vi "VIH UI - Append Control Rules.vi"(9 "Position Index (-1)":i32=-1, 10 "Ctrl Rules (new)":T1[](array[typedef]), 11 "Ctrl Rules (existing)":T1[](array[typedef])) -> (1 "Indices":i32[](array[numeric]), 3 "Ctrl Rules out":T1[](array[typedef]))   [LabVIEW 2014]
doc: "::: VI Helpeks :::\nCopyright (c) 2000-2026 Konstantin Shifershteyn. All rights reserved."
uses:
  _VIH HelpGen.llb/VIH HelpGen Typedef - Cluster - Control Rule.ctl
  _VIH HelpGen.llb/VIH HelpGen Typedef - Enum - Description Mode.ctl
  _VIH HelpGen.llb/VIH HelpGen Typedef - Enum - Default,Enable,Disable.ctl
  _VIH HelpGen.llb/VIH HelpGen Typedef - Cluster - Enum Value Info.ctl
panel:
  # "VI Helpeks\nCopyright (c) 2012-2026 Konstantin Shifershteyn"
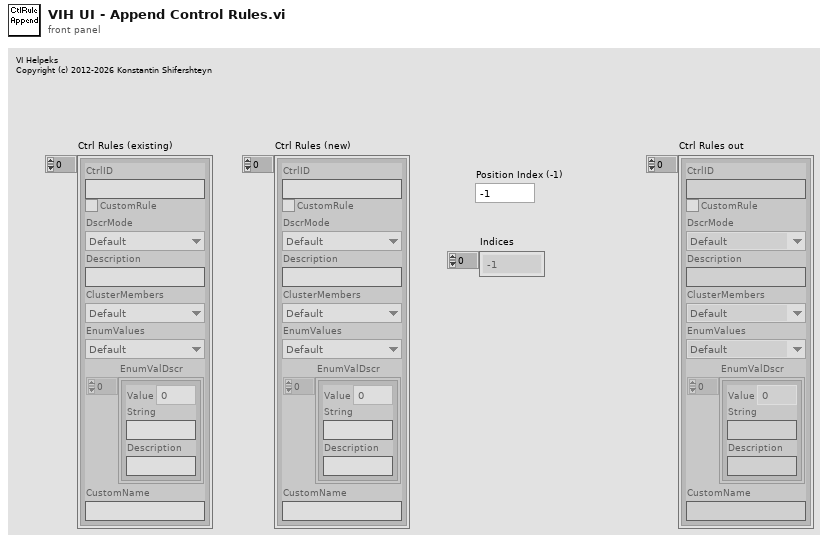
[diagram p1: front panel]
types:
  T1 = typedef "VIH HelpGen Typedef - Cluster - Control Rule.ctl" = cluster{"CtrlID":string, "CustomRule":bool, "DscrMode":T2, "Description":string, "ClusterMembers":T3, "EnumValues":T3, "EnumValDscr":T4[], "CustomName":string}
  T2 = typedef "VIH HelpGen Typedef - Enum - Description Mode.ctl" = enum16{"Default", "Description", "Description1", "Description2", "Custom", "None"}
  T3 = typedef "VIH HelpGen Typedef - Enum - Default,Enable,Disable.ctl" = enum16{"Default", "Enable", "Disable"}
  T4 = typedef "VIH HelpGen Typedef - Cluster - Enum Value Info.ctl" = cluster{"Value":ext, "String":string, "Description":string}
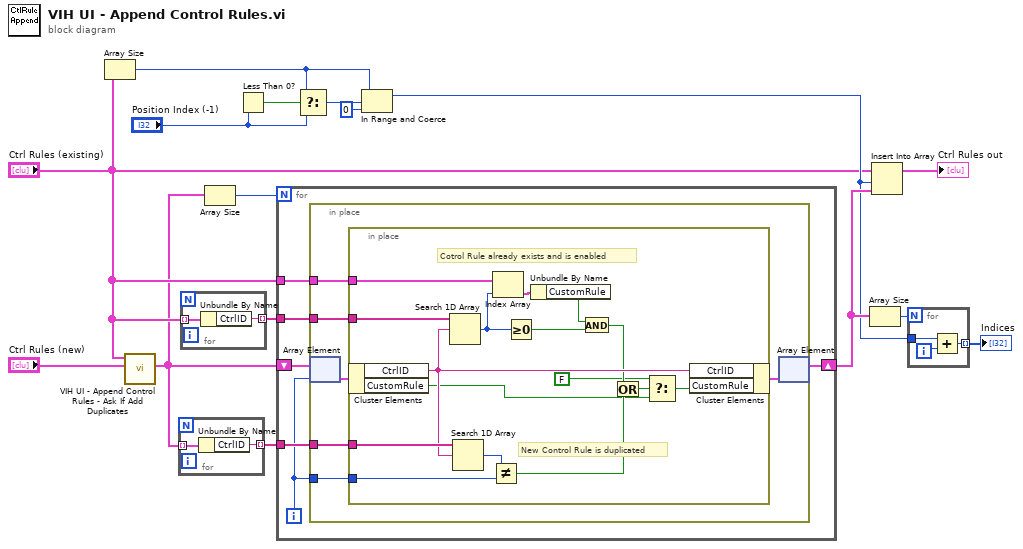
[diagram p0: block diagram]
diagram:
  n1 = Array Size(array="Ctrl Rules (existing)") -> (size(s)=w6:i32)
  n2 = call "VIH UI - Append Control Rules - Ask If Add Duplicates.vi"("Ctrl Rules (new)"="Ctrl Rules (new)", "Ctrl Rules (existing)"="Ctrl Rules (existing)") -> ("Ctrl Rules (new) out"=w1:T1[])  [unwired: 9 in]
  n3 = for {
    tunnel: w1 -> [w18] mode=indexing
    tunnel: [w17] -> w2 mode=indexing
    n4 = Unbundle By Name(w18) -> ("CtrlID"=w17:string)
  }
  n5 = for {
    tunnel: "Ctrl Rules (existing)" -> [w20] mode=indexing
    tunnel: [w19] -> w16 mode=indexing
    n6 = Unbundle By Name(w20) -> ("CtrlID"=w19:string)
  }
  n7 = Array Size(array=w1) -> (size(s)=w15:i32)
  n8 = Less Than 0?(x="Position Index (-1)") -> (x < 0?=w14:bool)
  n9 = for {
    N: w15 -> [_]
    tunnel: w16 -> [w25]
    shift-right: [w24] -> w9
    shift-left: w1 -> [w26]
    tunnel: "Ctrl Rules (existing)" -> [w23]
    tunnel: w2 -> [w22]
    i -> [w21]
    n10 = in-place {
      in-place-border: w25 -> [w30]
      in-place-border: w23 -> [w29]
      in-place-border: w22 -> [w28]
      in-place-border: w21 -> [w27]
      n11 = in-place-array #1(w26, w21) -> (w32:T1)
      n12 = in-place {
        in-place-border: w30 -> [w48]
        in-place-border: w29 -> [w47]
        in-place-border: w28 -> [w44]
        in-place-border: w27 -> [w41]
        # "New Control Rule is duplicated"
        # "Cotrol Rule already exists and is enabled"
        n13 = in-place-cluster #2(w32) -> ("CtrlID"=w43:string, "CustomRule"=w33:bool)
        n14 = Search 1D Array(1D array=w48, element=w43) -> (index of element=w40:i32)  [unwired: 1 in]
        n15 = Search 1D Array(1D array=w44, element=w43) -> (index of element=w42:i32)  [unwired: 1 in]
        n16 = Not Equal?(x=w42, y=w41) -> (x != y?=w36:bool)
        n17 = Index Array(array=w47, index=w40) -> (element=w46:T1)
        n18 = Greater Or Equal To 0?(x=w40) -> (x >= 0?=w39:bool)
        n19 = Unbundle By Name(w46) -> ("CustomRule"=w38:bool)
        n20 = And(x=w38, y=w39) -> (x .and. y?=w37:bool)
        n21 = Or(x=w37, y=w36) -> (x .or. y?=w35:bool)
        n22 = Select(t=FALSE ("f"), s=w35, f=w33) -> (s? t:f=w45:bool)
        n23 = in-place-cluster #2("CtrlID"=w43, "CustomRule"=w45) -> (w31:T1)
      }
      n24 = in-place-array #1(w31) -> (w24:T1[])  [unwired: 1 out]
    }
  }
  n25 = Select(t=w6, s=w14, f="Position Index (-1)") -> (s? t:f=w7:i32)
  n26 = In Range and Coerce(upper limit=w6, x=w7, lower limit=0) -> (coerced(x)=w8:i32)  [unwired: 1 out]
  n27 = Array Size(array=w9) -> (size(s)=w10:i32)
  n28 = Insert Into Array(array="Ctrl Rules (existing)", index=w8, new element=w9) -> (→"Ctrl Rules out":T1[])
  n29 = for {
    N: w10 -> [_]
    tunnel: w8 -> [w50]
    tunnel: [w49] -> w11 mode=indexing
    i -> [w51]
    n30 = Add(x=w50, y=w51) -> (x+y=w49:i32)
  }
  "Indices" <- w11
